vi "Regenerate gRPC code.vi"(11 "proto File Path":path) -> (0 "error out":errorcluster)   [LabVIEW 2021]
uses:
  <vilib>/CIF Foundation/CIF Plugin Wizard/Template Core Utilities/TemplateCoreUtilities.lvlib
panel:
  # "Instructions:\nIf run from the default location the proto file path can be left empty and it will auto-detect the path.  \nRun the VI.  It will attempt to generate and replace the existing gRPC server and client code.  \nA popup dialog will appear asking if an error was presented from the gRPC code generation and giving the opportunity to revert the code gen changes so repairs can be made to the proto file and the script can be attempted again."
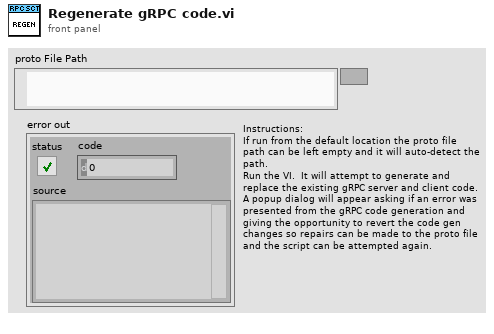
[diagram p1: front panel]
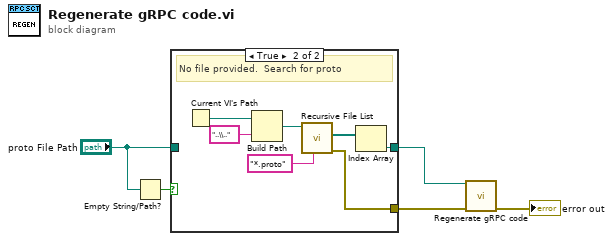
[diagram p0: block diagram]
diagram:
  n1 = Empty String/Path?(string/path="proto File Path") -> (empty?=w4:bool)
  n2 = case shown="True" w4 {
    tunnel: [_ w9] -> w3
    tunnel: [w6 w7] -> w2
    tunnel: "proto File Path" -> [w6 _]
    frame False {
      # "proto provided"
    }
    frame True {
      # "No file provided.  Search for proto"
      n3 = Current VI's Path() -> (path=w12:path)
      n4 = Build Path(base path=w12, name or relative path="..\\.." ("String")) -> (appended path=w11:path)
      n5 = call <vilib>:"Recursive File List.vi"("pattern"="*.proto", "Folder Path"=w11) -> ("error out"=w9:errorcluster, "All Files in Dir"=w8:path[])  [unwired: 5 in, 3 out]
      n6 = Index Array(array=w8) -> (element=w7:path)  [unwired: 1 in]
    }
  }
  n7 = call <vilib>:"Regenerate gRPC code.vi"("error in (no error)"=w3, "proto File Path"=w2) -> ("error out"=→"error out":errorcluster)  [unwired: 9 in]
